vi "Main.vi"() -> ()   [LabVIEW 2025]
uses:
  Controls/HR_Data_Structure.ctl
  Controls/Runners_Data.ctl
  Controls/Raw_Data.ctl
panel:
  in  "Wyjscie":path
  in  "Plik do analizy":path
  in  "HR Data Structure":T1={"Runners_Data"={"Name"="", "Age"=0}, "HR Max"=0, "Raw Data"={"Time"=[], "Bpm"=[]}, "% HR MAX"=[], "Total Time In Zone"=[], "Zones info"=[["Z1", "Endurance"], ["Z2", "Moderate"], ["Z3", "Tempo"], ["Z4", "Threshold"], ["Z5", "Anaerobic"]], "Heart Rate Zone No"=[]}
  out "HR":T1={"Runners_Data"={"Name"="", "Age"=0}, "HR Max"=0, "Raw Data"={"Time"=[], "Bpm"=[]}, "% HR MAX"=[], "Total Time In Zone"=[], "Zones info"=[["Z1", "Endurance"], ["Z2", "Moderate"], ["Z3", "Tempo"], ["Z4", "Threshold"], ["Z5", "Anaerobic"]], "Heart Rate Zone No"=[]}
  in  "Stop":bool
  in  "Save":bool
  in  "New Training":bool
  out "error out":errorcluster
  in  "error in":errorcluster
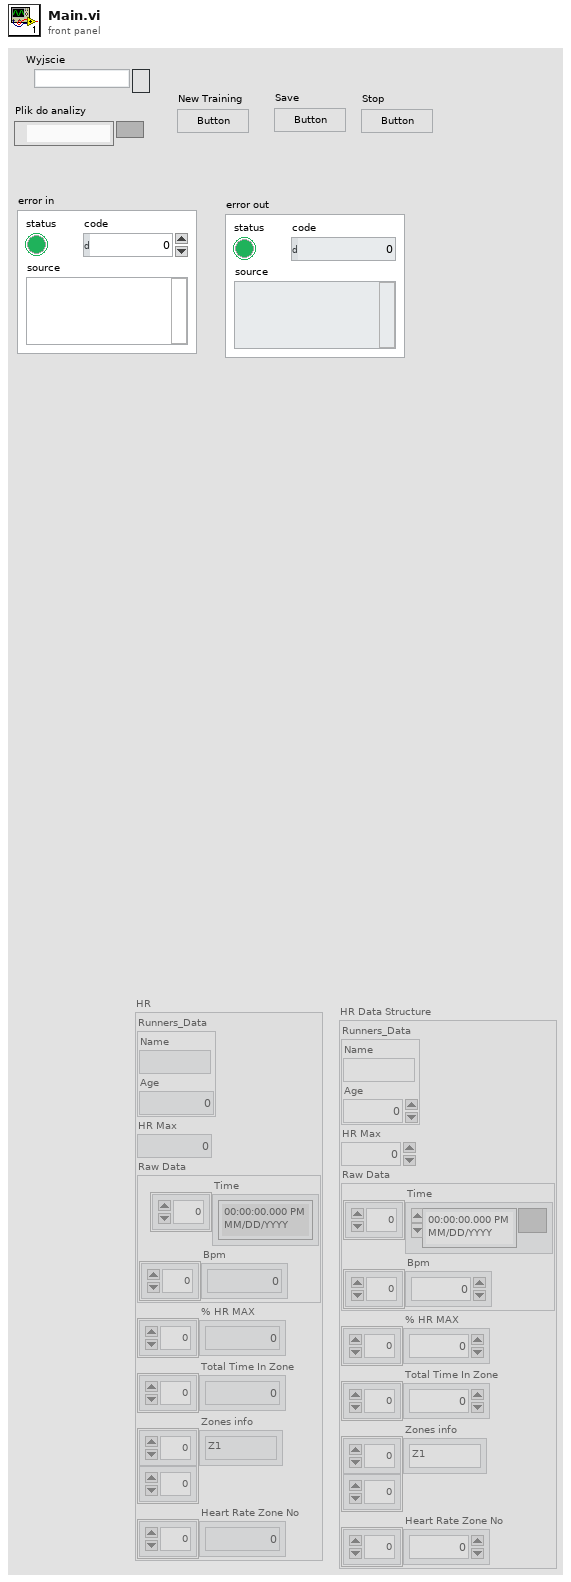
[diagram p1: front panel]
types:
  T1 = typedef "HR_Data_Structure.ctl" = cluster{"Runners_Data":T2, "HR Max":i32, "Raw Data":T3, "% HR MAX":dbl[], "Total Time In Zone":dbl[], "Zones info":string[][], "Heart Rate Zone No":dbl[]}
  T2 = typedef "Runners_Data.ctl" = cluster{"Name":string, "Age":i32}
  T3 = typedef "Raw_Data.ctl" = cluster{"Time":timestamp[], "Bpm":i32[]}
  T4 = enum16{"INIT", "IDLE", "SAVE", "ERROR", "NEW_TRAINING", "STOP"}
  T5 = enum16{"open", "replace", "create", "open or create", "replace or create", "replace or create with confirmation"}
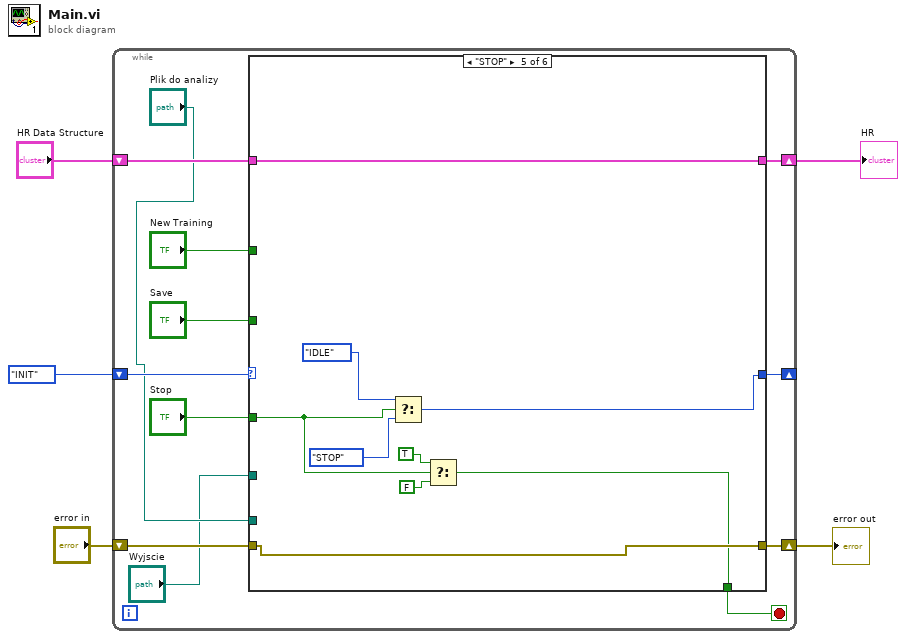
[diagram p0: block diagram]
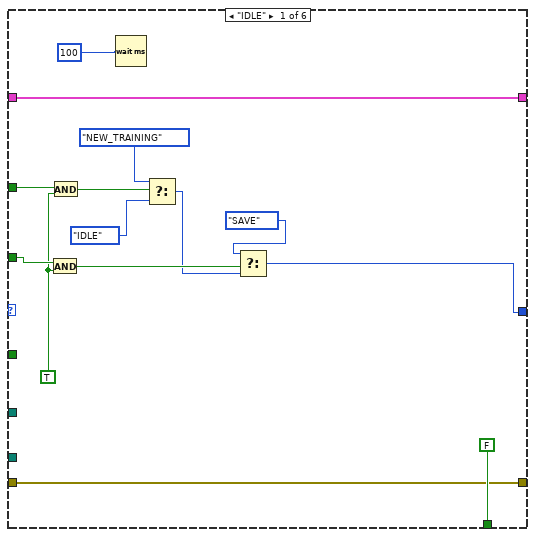
[diagram p2: hidden frame]
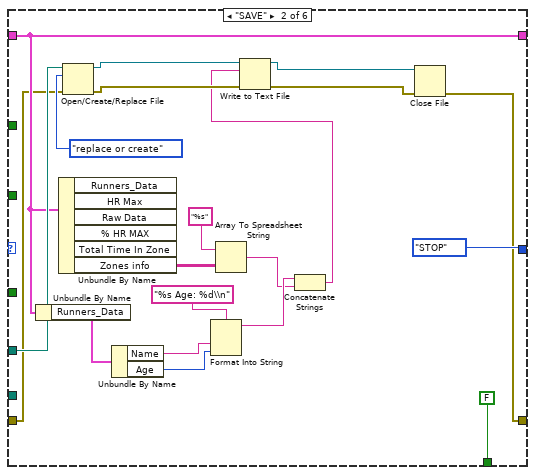
[diagram p3: hidden frame]
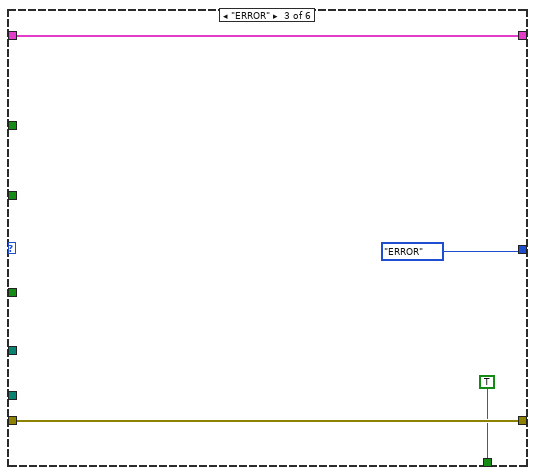
[diagram p4: hidden frame]
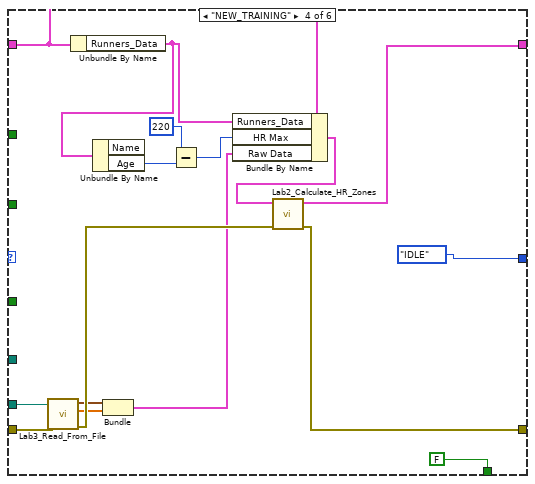
[diagram p5: hidden frame]
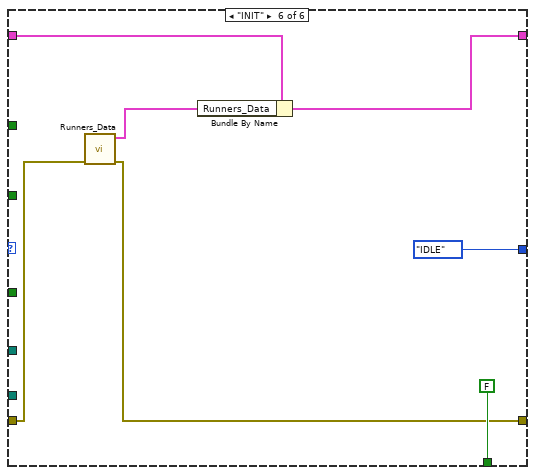
[diagram p6: hidden frame]
diagram:
  n1 = while {
    shift-right: [w16] -> w4
    shift-left: "error in" -> [w17]
    shift-right: [w14] -> _
    shift-left: T4."INIT" ("Enum") -> [w15]
    shift-right: [w11] -> w2
    shift-left: "HR Data Structure" -> [w12]
    stop <- w13 stop-if-true
    n2 = case shown="\"STOP\"" w15 {
      tunnel: w17 -> [w18 w41 w54 w71 w80 w84]
      tunnel: [w18 w38 w54 w69 w80 w83] -> w16
      tunnel: [w19 T4."STOP" ("Enum") T4."ERROR" ("Enum") T4."IDLE" ("Enum") w76 T4."IDLE" ("Enum")] -> w14
      tunnel: [FALSE FALSE TRUE FALSE w72 FALSE] -> w13
      tunnel: w12 -> [w31 w48 w55 w64 w79 w82]
      tunnel: [w31 w48 w55 w57 w79 w81] -> w11
      tunnel: "New Training" -> [w29 _ _ _ _ _]
      tunnel: "Save" -> [w28 _ _ _ _ _]
      tunnel: "Plik do analizy" -> [_ _ _ w67 _ _]
      tunnel: "Wyjscie" -> [_ w51 _ _ _ _]
      tunnel: "Stop" -> [_ _ _ _ w75 _]
      frame "IDLE" {
        w27 = TRUE ("y")
        n3 = And(x=w28, y=w27) -> (x .and. y?=w22:bool)
        n4 = And(x=w29, y=w27) -> (x .and. y?=w24:bool)
        n5 = Wait (ms)(milliseconds to wait=u32 100) -> ()  [unwired: 1 out]
        n6 = Select(t=T4."NEW_TRAINING", s=w24, f=T4."IDLE") -> (s? t:f=w20:T4)
        n7 = Select(t=T4."SAVE", s=w22, f=w20) -> (s? t:f=w19:T4)
      }
      frame "SAVE" {
        n8 = Unbundle By Name(w48) -> ("Runners_Data"=w46:T2)
        n9 = Unbundle By Name(w48) -> ("Zones info"=w35:string[][])  [unwired: 5 out]
        n10 = Open/Create/Replace File(file path (use dialog)=w51, error in=w41, operation (0:open)=T5."replace or create") -> (refnum out=w37:refnum<file>, error out=w40:errorcluster)  [unwired: 3 in, 1 out]
        n11 = Unbundle By Name(w46) -> ("Name"=w45:string, "Age"=w44:i32)
        n12 = Format Into String(format string="%s Age: %d\\n", w45, w44) -> (resulting string=w43:string)  [unwired: 2 in, 1 out]
        n13 = Array To Spreadsheet String(array=w35, 3:"%s" ("format string")) -> (spreadsheet string=w34:string)  [unwired: 1 in]
        n14 = Concatenate Strings(w43, w34) -> (w33:string)
        n15 = Write to Text File(file (use dialog)=w37, text=w33, error in=w40) -> (refnum out=w36:refnum<file>, error out=w39:errorcluster)  [unwired: 1 in, 1 out]
        n16 = Close File(refnum=w36, error in=w39) -> (error out=w38:errorcluster)  [unwired: 1 out]
      }
      frame "ERROR" {
      }
      frame "NEW_TRAINING" {
        n17 = call "Lab3_Read_From_File.vi"("error in"=w71, "File Path"=w67) -> ("error out"=w70:errorcluster, "Array"=w62:dbl[], "Array 2"=w61:timestamp[])  [unwired: 7 in]
        n18 = Unbundle By Name(w64) -> ("Runners_Data"=w59:T2)
        n19 = Unbundle By Name(w59) -> ("Age"=w66:i32)  [unwired: 1 out]
        n20 = Bundle("Array 2"=w61, "Array"=w62) -> (w60:cluster{"Array 2":timestamp[], "Array":dbl[]})  [unwired: 1 in]
        n21 = Subtract(x=220, y=w66) -> (x-y=w63:i32)
        n22 = Bundle By Name(cluster=w64, "Runners_Data"=w59, "HR Max"=w63, "Raw Data"=w60) -> (w58:T1)
        n23 = call "Lab2_Calculate_HR_Zones.vi"("error in (no error)"=w70, "HR_IN"=w58) -> ("error out"=w69:errorcluster, "HR_OUT"=w57:T1)  [unwired: 8 in]
      }
      frame "STOP" {
        n24 = Select(t=T4."IDLE", s=w75, f=T4."STOP") -> (s? t:f=w76:T4)
        n25 = Select(t=TRUE, s=w75, f=FALSE) -> (s? t:f=w72:bool)
      }
      frame "INIT" {
        n26 = call "Runners_Data.vi"("error in"=w84) -> ("error out"=w83:errorcluster, "Runners Data Out"=w87:T2)  [unwired: 9 in]
        n27 = Bundle By Name(cluster=w82, "Runners_Data"=w87) -> (w81:T1)
      }
    }
  }
  "error out" <- w4
  "HR" <- w2
